vi "Pre Launch Init.vi"(11 "Async Methods Actor in":refnum<class "Async Methods Actor.lvclass">) -> (0 "error out":errorcluster, 3 "Async Methods Actor out":refnum<class "Async Methods Actor.lvclass">)   [LabVIEW 2026, in "Async Methods Actor.lvlib" / "Async Methods Actor.lvclass"]
doc: "(<B>Filename</B>: Actor Framework.lvlib:Actor.lvclass:Pre Launch Init.vi)\n\nDefines behavior that occurs after the Launch Nested Actor method is invoked but before the actor's Actor Core method begins running.\n\nBy default, this method does nothing. A descendant class may override it to define behavior."
uses:
  Async Methods Actor.lvclass
  Async Methods Actor.lvclass/Async Methods Actor.ctl
  Async Message Execution Status Map.ctl
  Async Message Execution Status.ctl
  Async Methods Running.ctl
  VI Refnums Map.ctl
  VI Refnums Map Value.ctl
  Async Call Method.ctl
  VI Refnum Lifetime.ctl
  <vilib>/ActorFramework/Actor/Actor.lvclass
  Async Methods Actor Messages/Async Message/Async Message.lvclass
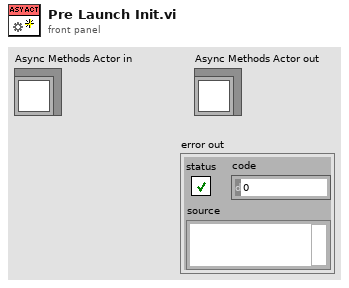
[diagram p1: front panel]
types:
  T1 = typedef "Async Methods Actor.lvlib/Async Methods Actor.lvclass/Async Message Execution Status Map.ctl" = map{string, T2}
  T2 = typedef "Async Methods Actor.lvlib/Async Methods Actor.lvclass/Async Message Execution Status.ctl" = cluster{"C&C Clones Running":u32, "C&F Clones Launched":u32}
  T3 = typedef "Async Methods Actor.lvlib/Async Methods Actor.lvclass/Async Methods Running.ctl" = cluster{"Async Messages":string[], "C&C Running":u32[], "C&F Launched":u32[]}
  T4 = typedef "Async Methods Actor.lvlib/Async Methods Actor.lvclass/VI Refnums Map.ctl" = map{refnum<vi>, T5}
  T5 = typedef "Async Methods Actor.lvlib/Async Methods Actor.lvclass/VI Refnums Map Value.ctl" = cluster{"Async Call Method":T6, "VI Refnum Lifecycle":T7, "Message Path":path}
  T6 = typedef "Async Methods Actor.lvlib/Async Methods Actor.lvclass/Async Call Method.ctl" = enum16{"Call and Collect", "Call and Forget"}
  T7 = typedef "Async Methods Actor.lvlib/Async Methods Actor.lvclass/VI Refnum Lifetime.ctl" = enum16{"Destroy on Exit", "Destroy on Actor Exit", "Destroy on Application Exit"}
  T8 = typedef "Async Methods Actor.lvlib/Async Methods Actor.lvclass/Running Methods Communication.ctl" = enum16{"None", "Notifier", "Event"}
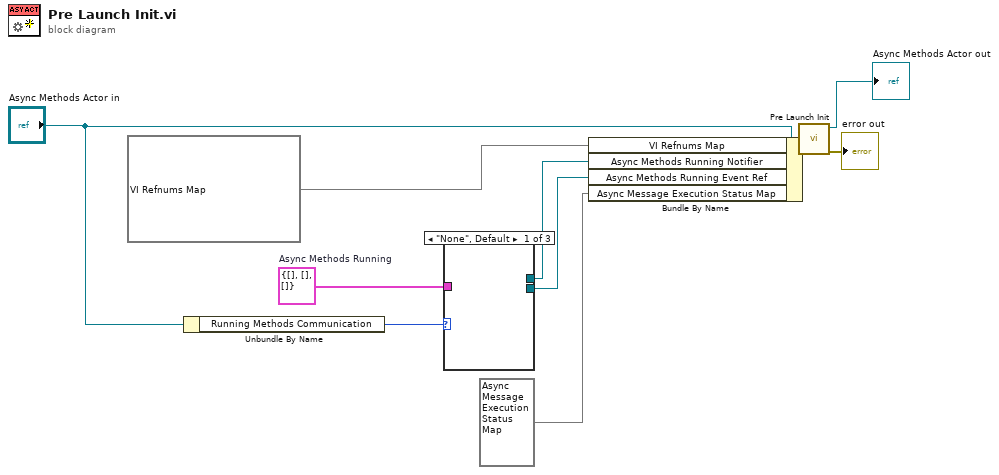
[diagram p0: block diagram]
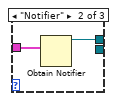
[diagram p2: hidden frame]
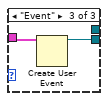
[diagram p3: hidden frame]
diagram:
  w7 = T3 {"Async Messages"=[], "C&C Running"=[], "C&F Launched"=[]}  # Async Methods Running
  n1 = Unbundle By Name("Async Methods Actor in") -> ("Running Methods Communication"=w3:T8)
  n2 = case shown="\"None\", Default" w3 {
    tunnel: w7 -> [_ w12 w14]
    tunnel: [_ w11 _] -> w6
    tunnel: [_ _ w13] -> w2
    frame "None", Default {
    }
    frame "Notifier" {
      n3 = Obtain Notifier(notification data type=w12) -> (notifier out=w11:refnum<notifier>)  [unwired: 3 in, 2 out]
    }
    frame "Event" {
      n4 = Create User Event(user event datatype=w14) -> (user event=w13:refnum<user-event>)  [unwired: 1 in, 1 out]
    }
  }
  n5 = Bundle By Name(cluster="Async Methods Actor in", "VI Refnums Map"=T4 {}, "Async Methods Running Notifier"=w6, "Async Methods Running Event Ref"=w2, "Async Message Execution Status Map"=T1 {} ("empty map")) -> (w9:refnum<class "Async Methods Actor.lvclass">)
  n6 = call-parent "Pre Launch Init.vi"("Actor in"=w9) -> ("error out"=→"error out":errorcluster, "Actor out"=→"Async Methods Actor out":refnum<class "Async Methods Actor.lvclass">)  [unwired: 9 in]
